vi "REST_Call.vi"(6 "timeout ms (5000)":i32=5000, 7 "method":T2, 8 "error in (no error)":errorcluster, 9 "body":string, 10 "url":string, 11 "client handle":T1) -> (0 "error out":errorcluster, 1 "response":string, 2 "status":i32, 3 "client handle out":T1)   [LabVIEW 2021, in "CANsub_Common.lvlib"]
doc: "Sends one HTTP request (GET, PUT, POST, DELETE) to the CANsub REST API and returns the HTTP status and the response body. An HTTP error status does not set error out: the caller must check status.\n\ntimeout ms: time limit for the complete request, default 5000"
uses:
  CANsub_Common.lvlib
  <vilib>/regexp/Match Regular Expression.xnode
  <vilib>/httpClient/LabVIEWHTTPClient.lvlib
  <vilib>/httpClient/PUTBuffer.vi
  <vilib>/httpClient/POSTBuffer.vi
  <vilib>/httpClient/ClientHandle.ctl
  Typedefs/HTTP_Method.ctl
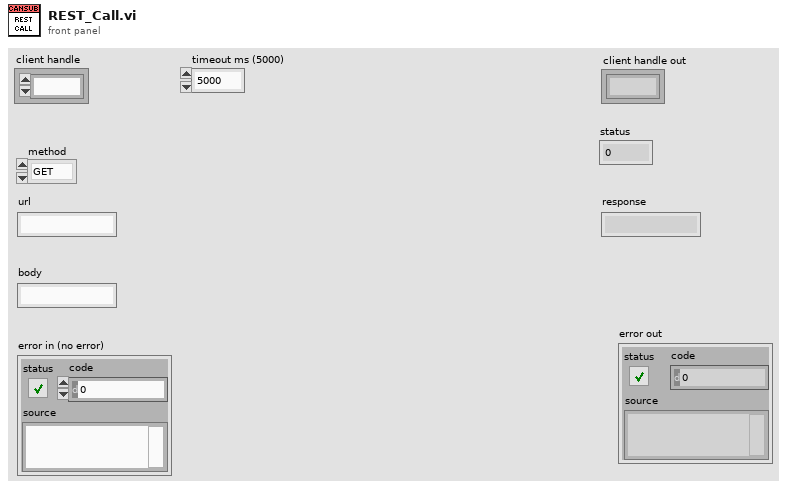
[diagram p1: front panel]
types:
  T1 = typedef "LabVIEWHTTPClient.lvlib/ClientHandle.ctl" = refnum<k1>
  T2 = typedef "CANsub_Common.lvlib/HTTP_Method.ctl" = enum16{"GET", "PUT", "POST", "DELETE"}
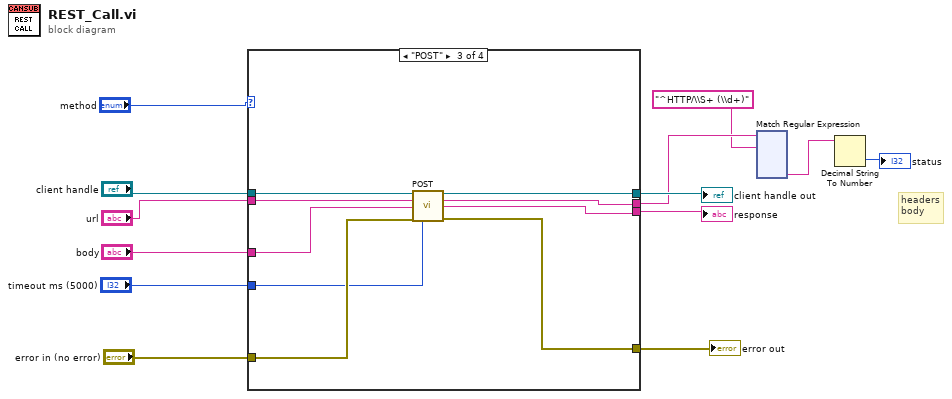
[diagram p0: block diagram]
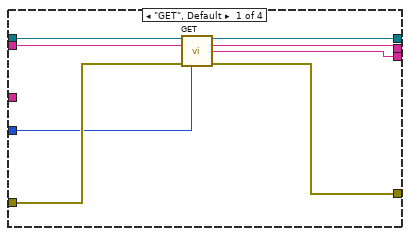
[diagram p2: hidden frame]
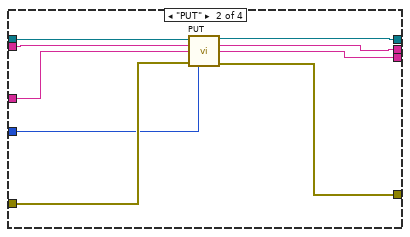
[diagram p3: hidden frame]
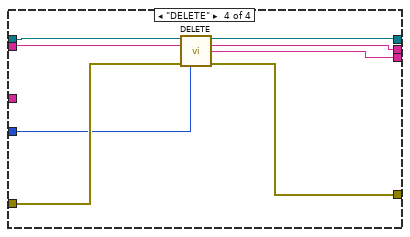
[diagram p4: hidden frame]
diagram:
  # "headers\nbody"
  n1 = case shown="\"POST\"" "method" {
    tunnel: "client handle" -> [w21 w30 w39 w47]
    tunnel: "url" -> [w20 w29 w38 w46]
    tunnel: "error in (no error)" -> [w19 w23 w33 w45]
    tunnel: [w18 w27 w36 w41] -> w8
    tunnel: [w17 w26 w35 w43] -> w5
    tunnel: [w16 w25 w34 w42] -> w7
    tunnel: [w15 w24 w32 w44] -> w6
    tunnel: "body" -> [_ w28 w37 _]
    tunnel: "timeout ms (5000)" -> [w14 w22 w31 w40]
    frame "GET", Default {
      n2 = call <vilib>:"GET.vi"("client handle"=w21, "url"=w20, "error in (no error)"=w19, "timeout (10000)"=w14) -> ("client handle out"=w18:T1, "headers"=w17:string, "body"=w16:string, "error out"=w15:errorcluster)  [unwired: 8 in]
    }
    frame "PUT" {
      n3 = call-poly <vilib>:"PUT.vi"("client handle"=w30, "url"=w29, "buffer"=w28, "error in (no error)"=w23, "timeout (10000)"=w22) -> ("client handle out"=w27:T1, "headers"=w26:string, "body"=w25:string, "error out"=w24:errorcluster)  [unwired: 7 in]
    }
    frame "POST" {
      n4 = call-poly <vilib>:"POST.vi"("client handle"=w39, "url"=w38, "buffer"=w37, "error in (no error)"=w33, "timeout (10000)"=w31) -> ("client handle out"=w36:T1, "headers"=w35:string, "body"=w34:string, "error out"=w32:errorcluster)  [unwired: 7 in]
    }
    frame "DELETE" {
      n5 = call <vilib>:"DELETE.vi"("client handle"=w47, "url"=w46, "error in (no error)"=w45, "timeout (10000)"=w40) -> ("client handle out"=w41:T1, "headers"=w43:string, "body"=w42:string, "error out"=w44:errorcluster)  [unwired: 8 in]
    }
  }
  "error out" <- w6
  "client handle out" <- w8
  "response" <- w7
  n6 = xnode "Match Regular Expression"("input string"=w5, "regular expression"="^HTTP/\\S+ (\\d+)") -> ("submatch 1"=w2:string)  [unwired: 4 in, 5 out]
  n7 = Decimal String To Number(string=w2) -> (number=→"status":i32)  [unwired: 2 in, 1 out]
